vi "Add Expectation.vi"(8 "error in (no error)":errorcluster, 10 "Expectations":refnum<class "Expectation.lvclass">, 11 "Mock in":refnum<class "LMock Mock.lvclass">) -> (0 "error out":errorcluster, 3 "Mock out":refnum<class "LMock Mock.lvclass">)   [LabVIEW 2020, in "LMock Mock.lvclass"]
uses:
  LMock Mock.lvclass
  Core/Expectation/Expectation.lvclass
  LMock Mock.lvclass/LMock Mock.ctl
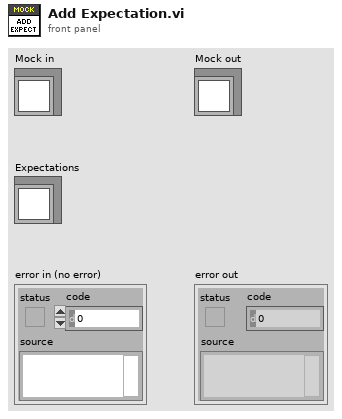
[diagram p1: front panel]
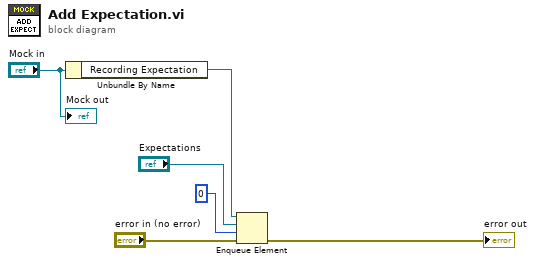
[diagram p0: block diagram]
diagram:
  n1 = Unbundle By Name("Mock in") -> ("Recording Expectation"=w3:refnum<queue>)
  n2 = Enqueue Element(queue=w3, element="Expectations", timeout in ms (-1)=0, error in (no error)="error in (no error)") -> (error out=→"error out":errorcluster)  [unwired: 2 out]
  "Mock out" <- "Mock in"
